vi "Untitled 7.vi"() -> ()   [LabVIEW 2026]
panel:
  out "Numeric 2":dbl
  in  "Numeric":dbl
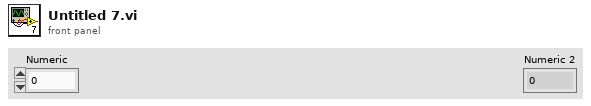
[diagram p1: front panel]
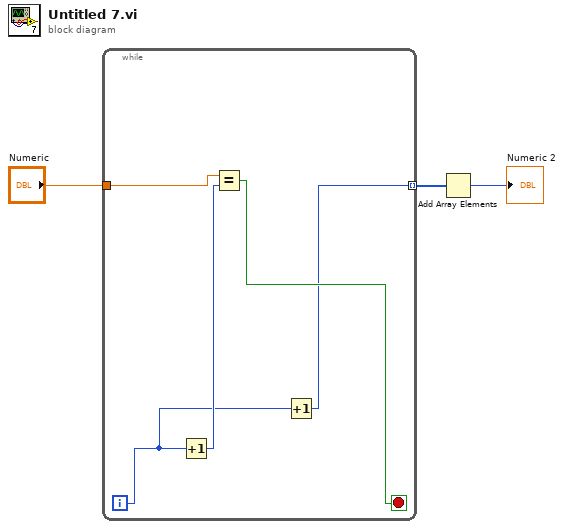
[diagram p0: block diagram]
diagram:
  n1 = while {
    tunnel: "Numeric" -> [w7]
    tunnel: [w5] -> w1 mode=indexing
    i -> [w4]
    stop <- w6 stop-if-true
    n2 = Increment(x=w4) -> (x+1=w8:i32)
    n3 = Equal?(x=w7, y=w8) -> (x = y?=w6:bool)
    n4 = Increment(x=w4) -> (x+1=w5:i32)
  }
  n5 = Add Array Elements(numeric array=w1) -> (sum=→"Numeric 2":i32)
